vi "Get Tag.vi"(5 "Override type":cluster{"ID":string, "Type":T1}, 7 "IFDO":T4(c390), 8 "error in 2":errorcluster, 9 "byte order (0:big-endian, network order)":T2(ring), 10 "Tag ID":T3=254 items=["NewSubfileType"=254, "ImageWidth"=256, "ImageLength"=257, "BitsPerSample"=258, "Compression"=259, "PhotometricInterpretation"=262, "StripOffsets"=273, "SamplesPerPixel"=277, "RowsPerStrip"=278, "StripByteCounts"=279, "XResolution"=282, "YResolution"=283, "ResolutionUnit"=296, "ColorMap"=320, "PlanarrConfiguration"=284, "YCbCrCoefficients"=529, "YCbCrSubSampling"=530, "YCbCrPositioning"=531, "ReferenceBlackWhite"=532, "BadFaxLines"=326, "CleanFaxData"=327, "ConsecutiveBadFaxLines"=328], 11 "File Refnum":refnum<file>) -> (0 "error out":errorcluster, 1 "Tag found?":bool, 2 "Data":variant, 3 "refnum out":refnum<file>)   [LabVIEW 2020, in "LV Tiff.lvlib"]
uses:
  LV Tiff.lvlib
  Tiff Data Type.ctl
  Tiff Tags.ctl
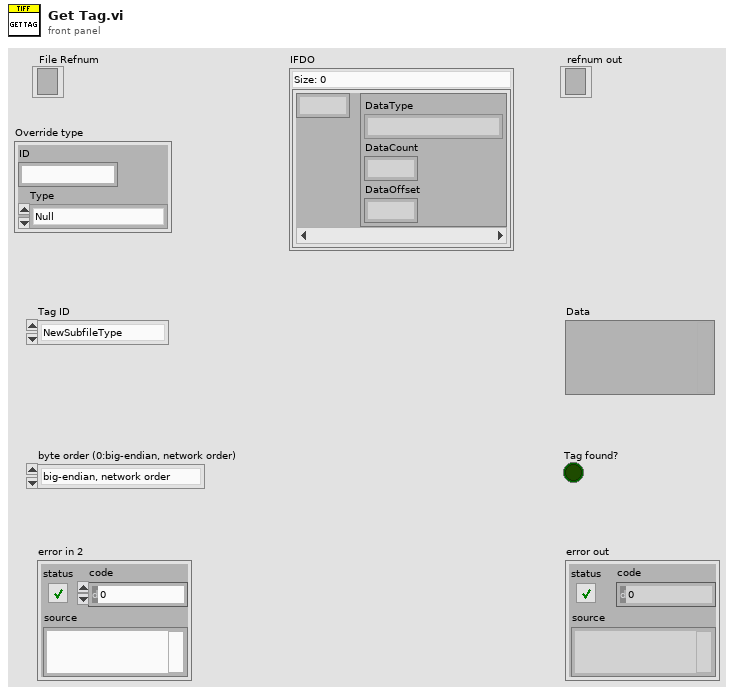
[diagram p1: front panel]
types:
  T1 = typedef "LV Tiff.lvlib/Tiff Data Type.ctl" = enum16{"Null", "BYTE", "ASCII", "SHORT", "LONG", "RATIONAL", "SBYTE", "UNDEFINE", "SSHORT", "SLONG", "SRATIONAL", "FLOAT", "DOUBLE"}
  T2 = enum16{"big-endian, network order", "native, host order", "little-endian"}
  T3 = typedef "LV Tiff.lvlib/Tiff Tags.ctl" = u16
  T4 = map{u16, cluster{"DataType":T1, "DataCount":u32, "DataOffset":u32}}
  T5 = cluster{"DataType":T1, "DataCount":u32, "DataOffset":u32}
  T6 = map{u16, cluster{"string array[0]":string, T1[]}}
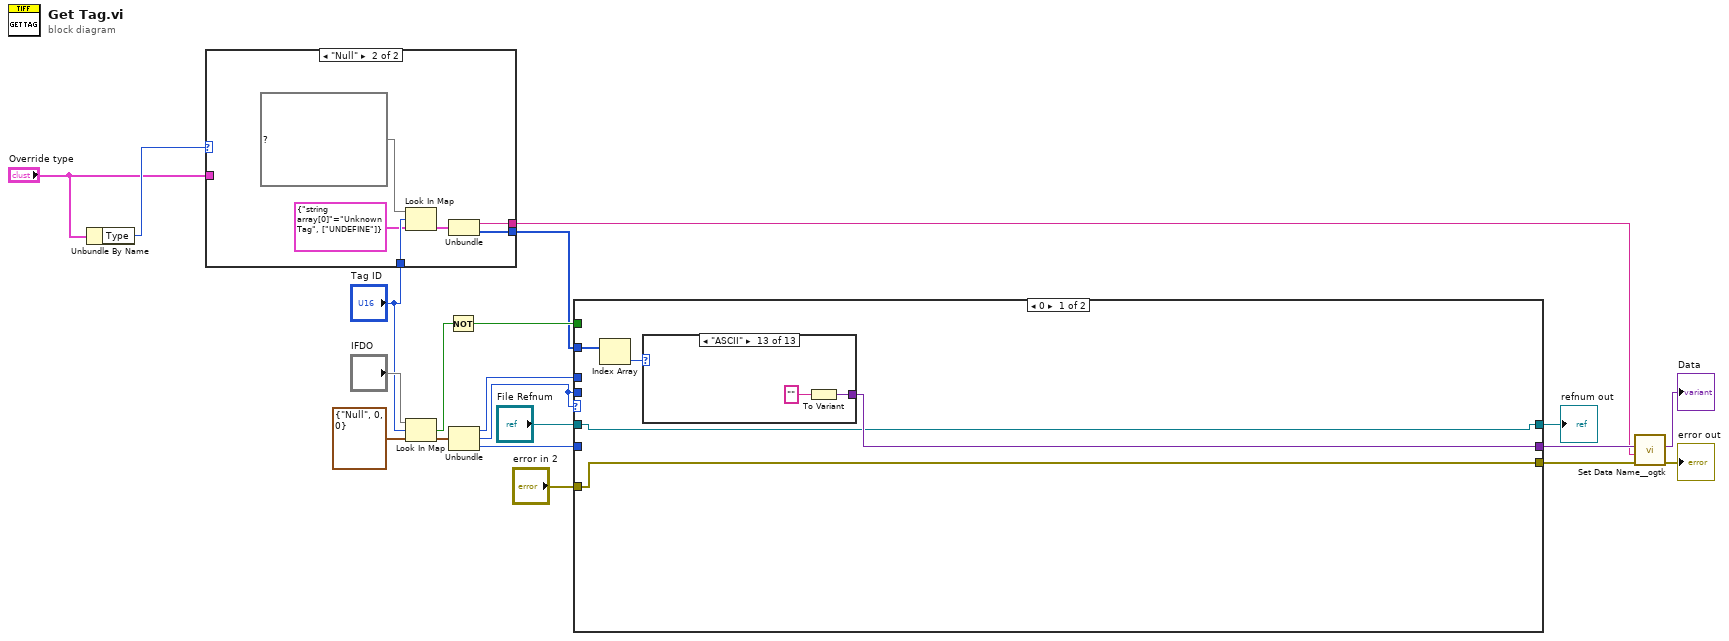
[diagram p0: block diagram]
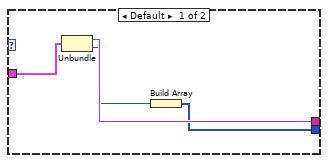
[diagram p2: hidden frame]
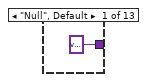
[diagram p3: hidden frame]
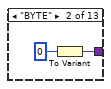
[diagram p4: hidden frame]
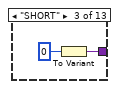
[diagram p5: hidden frame]
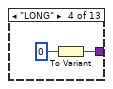
[diagram p6: hidden frame]
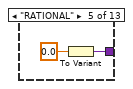
[diagram p7: hidden frame]
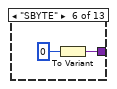
[diagram p8: hidden frame]
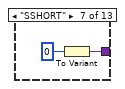
[diagram p9: hidden frame]
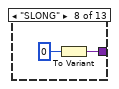
[diagram p10: hidden frame]
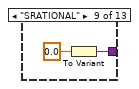
[diagram p11: hidden frame]
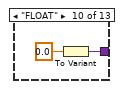
[diagram p12: hidden frame]
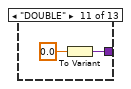
[diagram p13: hidden frame]
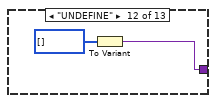
[diagram p14: hidden frame]
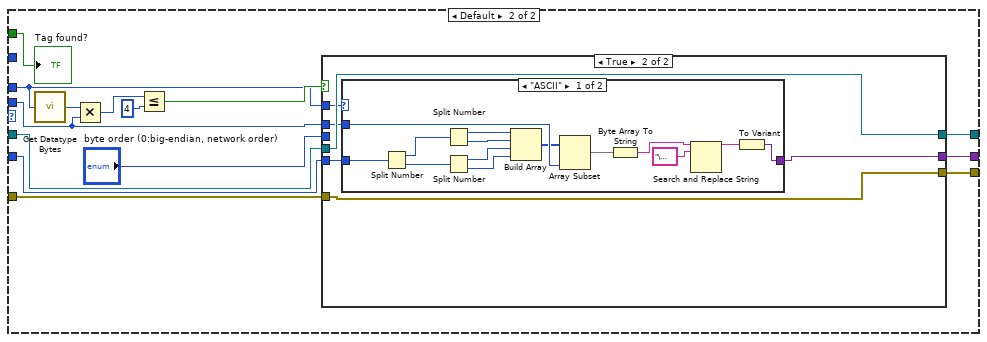
[diagram p15: hidden frame]
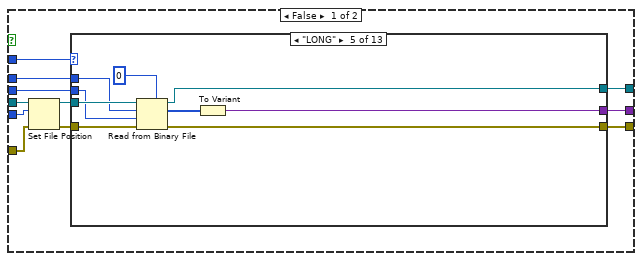
[diagram p16: hidden frame]
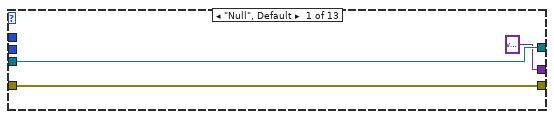
[diagram p17: hidden frame]
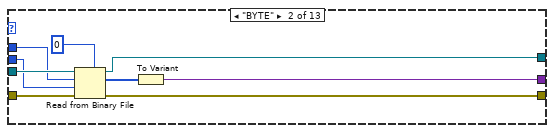
[diagram p18: hidden frame]
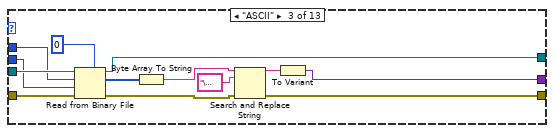
[diagram p19: hidden frame]
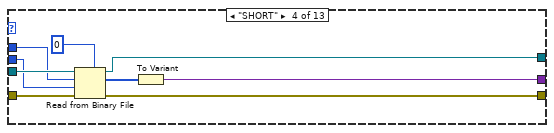
[diagram p20: hidden frame]
diagram:
  n1 = Unbundle By Name("Override type") -> ("Type"=w2:T1)
  n2 = case shown="\"Null\"" w2 {
    tunnel: "Tag ID" -> [_ w30]
    tunnel: [w23 w27] -> w7
    tunnel: [w21 w25] -> w5
    tunnel: "Override type" -> [w24 _]
    frame Default {
      n3 = Unbundle(w24) -> ("ID"=w23:string, "Type"=w22:T1)
      n4 = Build Array(w22) -> (w21:T1[])
    }
    frame "Null" {
      n5 = Look In Map(map=T6 {254={"string array[0]"="NewSubFileType", [enum."LONG"]}, 255={"string array[0]"="SubFileType", [enum."SHORT"]}, 256={"string array[0]"="ImageWidth", [enum."SHORT", enum."LONG"]}, 257={"string array[0]"="ImageHeight", [enum."SHORT", enum."LONG"]}, 258={"string array[0]"="BitsPerSample", [enum."SHORT"]}, 259={"string array[0]"="Compression", [enum."SHORT"]}, 262={"string array[0]"="PhotometricInterpretation", [enum."SHORT"]}, 263={"string array[0]"="Thresholding", [enum."SHORT"]}, 264={"string array[0]"="CellWidth", [enum."SHORT"]}, 265={"string array[0]"="CellLength", [enum."SHORT"]}, 266={"string array[0]"="FillOrder", [enum."SHORT"]}, 269={"string array[0]"="DocumentName", [enum."ASCII"]}, 270={"string array[0]"="ImageDescription", [enum."ASCII"]}, 271={"string array[0]"="Make", [enum."ASCII"]}, 272={"string array[0]"="Model", [enum."ASCII"]}, 273={"string array[0]"="StripOffsets", [enum."SHORT", enum."LONG"]}, 274={"string array[0]"="Orientation", [enum."SHORT"]}, 277={"string array[0]"="SamplesPerPixel", [enum."SHORT"]}, 278={"string array[0]"="RowsPerStrip", [enum."SHORT", enum."LONG"]}, 279={"string array[0]"="StripByteCounts", [enum."LONG", enum."SHORT"]}, 280={"string array[0]"="MinSampleValue", [enum."SHORT"]}, 281={"string array[0]"="MaxSampleValue", [enum."SHORT"]}, 282={"string array[0]"="XResolution", [enum."RATIONAL"]}, 283={"string array[0]"="YResolution", [enum."RATIONAL"]}, 284={"string array[0]"="PlanarConfiguration", [enum."SHORT"]}, 285={"string array[0]"="PageName", [enum."ASCII"]}, 286={"string array[0]"="XPosition", [enum."RATIONAL"]}, 287={"string array[0]"="YPosition", [enum."RATIONAL"]}, 288={"string array[0]"="FreeOffsets", [enum."LONG"]}, 289={"string array[0]"="FreeByteCounts", [enum."LONG"]}, 290={"string array[0]"="GrayResponseUnit", [enum."SHORT"]}, 291={"string array[0]"="GrayResponseCurve", [enum."SHORT"]}, 292={"string array[0]"="T4Options[2]", [enum."LONG"]}, 293={"string array[0]"="T6Options[3]", [enum."LONG"]}, 296={"string array[0]"="ResolutionUnit", [enum."SHORT"]}, 297={"string array[0]"="PageNumber", [enum."SHORT"]}, 300={"string array[0]"="ColorResponseUnit", [enum."SHORT"]}, 301={"string array[0]"="TransferFunction[4]", [enum."SHORT"]}, 305={"string array[0]"="Software", [enum."ASCII"]}, 306={"string array[0]"="DateTime", [enum."ASCII"]}, 315={"string array[0]"="Artist", [enum."ASCII"]}, 316={"string array[0]"="HostComputer", [enum."ASCII"]}, 317={"string array[0]"="Predictor", [enum."SHORT"]}, 318={"string array[0]"="WhitePoint", [enum."RATIONAL"]}, 319={"string array[0]"="PrimaryChromaticities", [enum."RATIONAL"]}, 320={"string array[0]"="ColorMap", [enum."SHORT"]}, 321={"string array[0]"="HalftoneHints", [enum."SHORT"]}, 322={"string array[0]"="TileWidth", [enum."SHORT", enum."LONG"]}, 323={"string array[0]"="TileLength", [enum."SHORT", enum."LONG"]}, 324={"string array[0]"="TileOffsets", [enum."LONG"]}, 325={"string array[0]"="TileByteCounts", [enum."SHORT", enum."LONG"]}, 326={"string array[0]"="BadFaxLines", [enum."SHORT", enum."LONG"]}, 327={"string array[0]"="CleanFaxData", [enum."SHORT"]}, 328={"string array[0]"="ConsecutiveBadFaxLines", [enum."LONG", enum."SHORT"]}, 332={"string array[0]"="InkSet", [enum."SHORT"]}, 333={"string array[0]"="InkNames", [enum."ASCII"]}, 334={"string array[0]"="NumberOfInks", [enum."SHORT"]}, 336={"string array[0]"="DotRange", [enum."BYTE", enum."SHORT"]}, 337={"string array[0]"="TargetPrinter", [enum."ASCII"]}, 338={"string array[0]"="ExtraSamples", [enum."BYTE"]}, 339={"string array[0]"="SampleFormat", [enum."SHORT"]}, 340={"string array[0]"="SMinSampleValue", [enum."Null"]}, 341={"string array[0]"="SMaxSampleValue", [enum."Null"]}, 342={"string array[0]"="TransferRange", [enum."SHORT"]}, 512={"string array[0]"="JPEGProc", [enum."SHORT"]}, 513={"string array[0]"="JPEGInterchangeFormat", [enum."LONG"]}, 514={"string array[0]"="JPEGInterchangeFormatLength", [enum."LONG"]}, 515={"string array[0]"="JPEGRestartInterval", [enum."SHORT"]}, 517={"string array[0]"="JPEGLosslessPredictors", [enum."SHORT"]}, 518={"string array[0]"="JPEGPointTransforms", [enum."SHORT"]}, 519={"string array[0]"="JPEGQTables", [enum."LONG"]}, 520={"string array[0]"="JPEGDCTTables", [enum."LONG"]}, 521={"string array[0]"="JPEGACTTables", [enum."LONG"]}, 529={"string array[0]"="YCbCrCoefficients", [enum."RATIONAL"]}, 530={"string array[0]"="YCbCrSubSampling", [enum."SHORT"]}, 531={"string array[0]"="YCbCrPositioning", [enum."SHORT"]}, 532={"string array[0]"="ReferenceBlackWhite", [enum."LONG"]}, 33432={"string array[0]"="Copyright", [enum."ASCII"]}} ("Map 2"), key=w30, default value=cluster{"string array[0]":string, T1[]} {"string array[0]"="Unknown Tag", [enum."UNDEFINE"]}) -> (value=w29:cluster{"string array[0]":string, T1[]})  [unwired: 1 out]
      n6 = Unbundle(w29) -> ("string array[0]"=w27:string, w25:T1[])
    }
  }
  n7 = Look In Map(map="IFDO", key="Tag ID", default value=T5 {"DataType"=enum."Null", "DataCount"=0, "DataOffset"=0}) -> (key not found?=w15:bool, value=w19:T5)
  n8 = Not(x=w15) -> (.not. x?=w16:bool)
  n9 = Unbundle(w19) -> ("DataType"=w13:T1, "DataCount"=w6:u32, "DataOffset"=w14:u32)
  n10 = case shown="0" w6 {
    tunnel: [w32 w74] -> w18
    tunnel: [w31 w73] -> w17
    tunnel: w16 -> [_ w72]
    tunnel: w14 -> [_ w66]
    tunnel: w13 -> [_ w65]
    tunnel: w6 -> [_ w64]
    tunnel: [w33 w63] -> w10
    tunnel: w5 -> [w35 _]
    tunnel: "File Refnum" -> [w32 w62]
    tunnel: "error in 2" -> [w31 w61]
    frame 0 {
      n11 = Index Array(array=w35) -> (element=w34:T1)  [unwired: 1 in]
      n12 = case shown="\"ASCII\"" w34 {
        tunnel: [variant ("Variant") w37 w39 w41 w43 w45 w47 w49 w51 w53 w55 w57 w59] -> w33
        frame "Null", Default {
        }
        frame "BYTE" {
          n13 = To Variant(anything=u8 0) -> (Variant=w37:variant)
        }
        frame "SHORT" {
          n14 = To Variant(anything=u16 0) -> (Variant=w39:variant)
        }
        frame "LONG" {
          n15 = To Variant(anything=u32 0) -> (Variant=w41:variant)
        }
        frame "RATIONAL" {
          n16 = To Variant(anything=0.0) -> (Variant=w43:variant)
        }
        frame "SBYTE" {
          n17 = To Variant(anything=i8 0) -> (Variant=w45:variant)
        }
        frame "SSHORT" {
          n18 = To Variant(anything=i16 0) -> (Variant=w47:variant)
        }
        frame "SLONG" {
          n19 = To Variant(anything=0) -> (Variant=w49:variant)
        }
        frame "SRATIONAL" {
          n20 = To Variant(anything=0.0) -> (Variant=w51:variant)
        }
        frame "FLOAT" {
          n21 = To Variant(anything=sgl 0.0) -> (Variant=w53:variant)
        }
        frame "DOUBLE" {
          n22 = To Variant(anything=0.0) -> (Variant=w55:variant)
        }
        frame "UNDEFINE" {
          n23 = To Variant(anything=u8[] []) -> (Variant=w57:variant)
        }
        frame "ASCII" {
          n24 = To Variant(anything="") -> (Variant=w59:variant)
        }
      }
    }
    frame Default {
      n25 = call "Get Datatype Bytes.vi"("DataType"=w65) -> ("N Bytes"=w70:u8)
      n26 = Multiply(x=w70, y=w64) -> (x*y=w69:u32)
      n27 = Less Or Equal?(x=w69, y=u32 4) -> (x <= y?=w67:bool)
      n28 = case shown="True" w67 {
        tunnel: [w75 w224] -> w63
        tunnel: w66 -> [w79 w225]
        tunnel: w62 -> [w85 w229]
        tunnel: [w83 w229] -> w74
        tunnel: w61 -> [w82 w228]
        tunnel: [w80 w228] -> w73
        tunnel: w65 -> [w78 w226]
        tunnel: w64 -> [w77 w227]
        tunnel: "byte order (0:big-endian, network order)" -> [w76 _]
        frame False {
          n29 = Set File Position(offset (in bytes) (0)=w79, refnum=w85, error in=w82) -> (refnum out=w84:refnum<file>, error out=w81:errorcluster)  [unwired: 1 in]
          n30 = case shown="\"LONG\"" w78 {
            tunnel: w84 -> [w88 w97 w110 w119 w128 w140 w157 w166 w175 w184 w193 w202 w215]
            tunnel: [w88 w96 w109 w118 w127 w139 w156 w165 w174 w183 w192 w201 w214] -> w83
            tunnel: w81 -> [w86 w95 w108 w117 w126 w138 w155 w164 w173 w182 w191 w200 w213]
            tunnel: [w86 w94 w99 w116 w125 w137 w154 w163 w172 w181 w190 w199 w212] -> w80
            tunnel: w77 -> [_ w92 w106 w114 w123 w131 w153 w162 w171 w180 w189 w198 w205]
            tunnel: w76 -> [_ w91 w105 w113 w122 w136 w152 w161 w170 w179 w188 w197 w211]
            tunnel: [variant ("Variant") w89 w103 w112 w121 w135 w151 w160 w169 w178 w187 w196 w210] -> w75
            frame "Null", Default {
            }
            frame "BYTE" {
              n31 = Read from Binary File(5:u8 0, 8:w95, 9:w91, 10:w92, 11:w97) -> (0:w94:errorcluster, 2:w90:u8[], 3:w96:refnum<file>)  [unwired: 1 in, 1 out]
              n32 = To Variant(anything=w90) -> (Variant=w89:variant)
            }
            frame "ASCII" {
              n33 = Read from Binary File(5:u8 0, 8:w108, 9:w105, 10:w106, 11:w110) -> (0:w100:errorcluster, 2:w104:u8[], 3:w109:refnum<file>)  [unwired: 1 in, 1 out]
              n34 = Byte Array To String(unsigned byte array=w104) -> (string=w102:string)
              n35 = Search and Replace String(input string=w102, search string="\u0000", error in=w100) -> (result string=w101:string, error out=w99:errorcluster)  [unwired: 5 in, 2 out]
              n36 = To Variant(anything=w101) -> (Variant=w103:variant)
            }
            frame "SHORT" {
              n37 = Read from Binary File(5:u16 0, 8:w117, 9:w113, 10:w114, 11:w119) -> (0:w116:errorcluster, 2:w111:u16[], 3:w118:refnum<file>)  [unwired: 1 in, 1 out]
              n38 = To Variant(anything=w111) -> (Variant=w112:variant)
            }
            frame "LONG" {
              n39 = Read from Binary File(5:u32 0, 8:w126, 9:w122, 10:w123, 11:w128) -> (0:w125:errorcluster, 2:w120:u32[], 3:w127:refnum<file>)  [unwired: 1 in, 1 out]
              n40 = To Variant(anything=w120) -> (Variant=w121:variant)
            }
            frame "RATIONAL" {
              n41 = Read from Binary File(5:cluster{u32, u32} {0, 0}, 8:w138, 9:w136, 10:w131, 11:w140) -> (0:w137:errorcluster, 2:w133:cluster{u32, u32}[], 3:w139:refnum<file>)  [unwired: 1 in, 1 out]
              n42 = for {
                tunnel: w133 -> [w148] mode=indexing
                tunnel: [w145] -> w132 mode=indexing
                n43 = Unbundle(w148) -> (w147:u32, w146:u32)
                n44 = Divide(x=w147, y=w146) -> (x/y=w145:dbl)
              }
              n45 = Equal?(x=w131, y=u32 1) -> (x = y?=w129:bool)
              n46 = case shown="True" w129 {
                tunnel: [w142 w143] -> w135
                tunnel: w132 -> [w141 w144]
                frame False {
                  n47 = To Variant(anything=w141) -> (Variant=w142:variant)
                }
                frame True {
                  n48 = Index Array(array=w144) -> (element=w143:dbl)  [unwired: 1 in]
                }
              }
            }
            frame "SBYTE" {
              n49 = Read from Binary File(5:i8 0, 8:w155, 9:w152, 10:w153, 11:w157) -> (0:w154:errorcluster, 2:w150:i8[], 3:w156:refnum<file>)  [unwired: 1 in, 1 out]
              n50 = To Variant(anything=w150) -> (Variant=w151:variant)
            }
            frame "UNDEFINE" {
              n51 = Read from Binary File(5:u8 0, 8:w164, 9:w161, 10:w162, 11:w166) -> (0:w163:errorcluster, 2:w159:u8[], 3:w165:refnum<file>)  [unwired: 1 in, 1 out]
              n52 = To Variant(anything=w159) -> (Variant=w160:variant)
            }
            frame "SSHORT" {
              n53 = Read from Binary File(5:i16 0, 8:w173, 9:w170, 10:w171, 11:w175) -> (0:w172:errorcluster, 2:w168:i16[], 3:w174:refnum<file>)  [unwired: 1 in, 1 out]
              n54 = To Variant(anything=w168) -> (Variant=w169:variant)
            }
            frame "SLONG" {
              n55 = Read from Binary File(5:0, 8:w182, 9:w179, 10:w180, 11:w184) -> (0:w181:errorcluster, 2:w177:i32[], 3:w183:refnum<file>)  [unwired: 1 in, 1 out]
              n56 = To Variant(anything=w177) -> (Variant=w178:variant)
            }
            frame "FLOAT" {
              n57 = Read from Binary File(5:sgl 0.0, 8:w191, 9:w188, 10:w189, 11:w193) -> (0:w190:errorcluster, 2:w186:sgl[], 3:w192:refnum<file>)  [unwired: 1 in, 1 out]
              n58 = To Variant(anything=w186) -> (Variant=w187:variant)
            }
            frame "DOUBLE" {
              n59 = Read from Binary File(5:0.0, 8:w200, 9:w197, 10:w198, 11:w202) -> (0:w199:errorcluster, 2:w195:dbl[], 3:w201:refnum<file>)  [unwired: 1 in, 1 out]
              n60 = To Variant(anything=w195) -> (Variant=w196:variant)
            }
            frame "SRATIONAL" {
              n61 = Read from Binary File(5:cluster{i32, i32} {0, 0}, 8:w213, 9:w211, 10:w205, 11:w215) -> (0:w212:errorcluster, 2:w208:cluster{i32, i32}[], 3:w214:refnum<file>)  [unwired: 1 in, 1 out]
              n62 = for {
                tunnel: w208 -> [w223] mode=indexing
                tunnel: [w220] -> w207 mode=indexing
                n63 = Unbundle(w223) -> (w222:i32, w221:i32)
                n64 = Divide(x=w222, y=w221) -> (x/y=w220:dbl)
              }
              n65 = Equal?(x=w205, y=u32 1) -> (x = y?=w203:bool)
              n66 = case shown="True" w203 {
                tunnel: [w217 w218] -> w206
                tunnel: w207 -> [w216 w219]
                frame False {
                  n67 = To Variant(anything=w216) -> (Variant=w217:variant)
                }
                frame True {
                  n68 = Index Array(array=w219) -> (element=w218:dbl)  [unwired: 1 in]
                }
              }
              n69 = To Variant(anything=w206) -> (Variant=w210:variant)
            }
          }
        }
        frame True {
          n70 = case shown="\"ASCII\"" w226 {
            tunnel: w227 -> [w242 _]
            tunnel: w225 -> [w243 w245]
            tunnel: [w241 w244] -> w224
            frame "ASCII" {
              n71 = Split Number(x=w243) -> (hi(x)=w240:u16, lo(x)=w239:u16)
              n72 = Split Number(x=w240) -> (hi(x)=w238:u8, lo(x)=w237:u8)
              n73 = Split Number(x=w239) -> (hi(x)=w236:u8, lo(x)=w235:u8)
              n74 = Build Array(w238, w237, w236, w235) -> (w234:u8[])
              n75 = Array Subset(array=w234, length=w242) -> (w233:u8[])  [unwired: 1 in]
              n76 = Byte Array To String(unsigned byte array=w233) -> (string=w232:string)
              n77 = Search and Replace String(input string=w232, search string="\u0000") -> (result string=w231:string)  [unwired: 6 in, 3 out]
              n78 = To Variant(anything=w231) -> (Variant=w241:variant)
            }
            frame Default {
              n79 = To Variant(anything=w245) -> (Variant=w244:variant)
            }
          }
        }
      }
      "Tag found?" <- w72
    }
  }
  "refnum out" <- w18
  n80 = call <userlib>:"Set Data Name__ogtk.vi"("error in (no error)"=w17, "Data Name"=w7, "Data"=w10) -> ("error out"=→"error out":errorcluster, "Renamed Data"=→"Data":variant)  [unwired: 7 in]
